vi "KYFG Get XML.vi"(0 "camHandle":u32, 9 "bufferSize":u64, 11 "error in (no error)":errorcluster) -> (4 "camHandle out":u32, 6 "buffer":u8[](array[numeric]), 8 "isZipFile":u8, 10 "bufferSize out":u64, 15 "error out":errorcluster)   [LabVIEW 2023, in "KYFGLib_lv.lvlib"]
doc: "KYFG_API FGSTATUS KYFG_GetXML(CAMHANDLE camHandle, char** buffer, unsigned long long *bufferSize, KYBOOL *isZipFile);"
uses:
  KYFGLib_lv.lvlib
  KYFGLib.dll
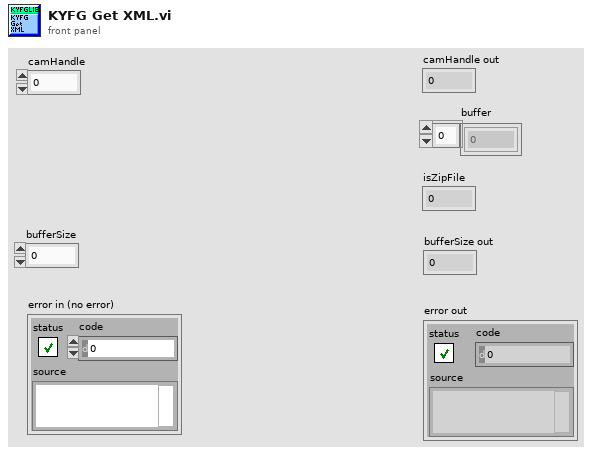
[diagram p1: front panel]
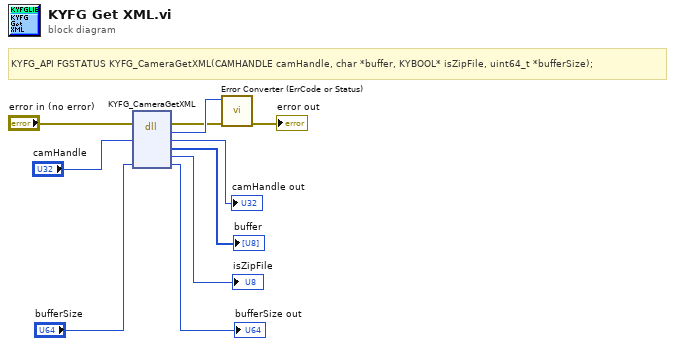
[diagram p0: block diagram]
diagram:
  # "KYFG_API FGSTATUS KYFG_CameraGetXML(CAMHANDLE camHandle, char *buffer, KYBOOL* isZipFile, uint64_t *bufferSize);"
  n1 = dll-call lib="KYFGLib.dll" fn="KYFG_CameraGetXML"(error in="error in (no error)", "camHandle"="camHandle", "bufferSize"="bufferSize") -> (error out=w7:errorcluster, "return type"=w10:u32, "camHandle"=→"camHandle out":u32, "buffer"=→"buffer":u8[], "isZipFile"=→"isZipFile":u8, "bufferSize"=→"bufferSize out":u64)  [unwired: 4 in, 1 out]
  n2 = call "Error Converter (ErrCode or Status).vi"("error in (no error)"=w7, "error code"=w10) -> ("error out"=→"error out":errorcluster)  [unwired: 9 in]
